vi "From CSV File.vi"(8 "error in (no error)":errorcluster, 9 "Path":path, 10 "engine in":refnum<class "engine configuration.lvclass">, 11 "Scan Engine editor node in":refnum<class "Scan Engine editor node.lvclass">) -> (0 "error out":errorcluster, 1 "Update":bool, 2 "engine out":refnum<class "engine configuration.lvclass">, 3 "Scan Engine editor node out":refnum<class "Scan Engine editor node.lvclass">)   [LabVIEW 2015, in "Scan Engine editor node.lvclass"]
uses:
  Scan Engine editor node.lvclass
  <vilib>/NI/Module Execution Interface/Engine Configuration/engine configuration.lvclass
  configuration/Scan Engine configuration.lvclass
  <vilib>/NI/Configuration Framework/serializable configuration/NISE_CEF_serializable configuration.lvclass/NISE_CEF_serializable configuration.ctl
  configuration/Scan Engine configuration.lvclass/Scan Engine configuration.ctl
  <vilib>/NI/Tag Bus/tag/tag descriptor.lvclass/tag descriptor.ctl
  <vilib>/Utility/LVClass/Get LV Class Name.vi
  <vilib>/NI/Configuration Framework/error generator/NISE_error generator.vi
  <vilib>/NI/Tag Bus Module Framework/channel/TBM channel.lvclass
  <vilib>/NI/Configuration Framework/serializable configuration/NISE_CEF_serializable configuration.lvclass
  <vilib>/NI/Tag Bus/tag/tag descriptor.lvclass
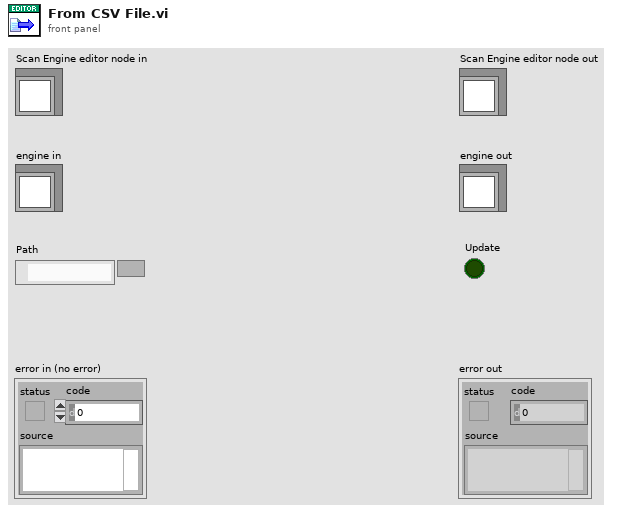
[diagram p1: front panel]
types:
  T1 = typedef "Scan Engine configuration.lvclass/Line.ctl" = cluster{"channel":refnum<class "TBM channel.lvclass">, "Tag":string}
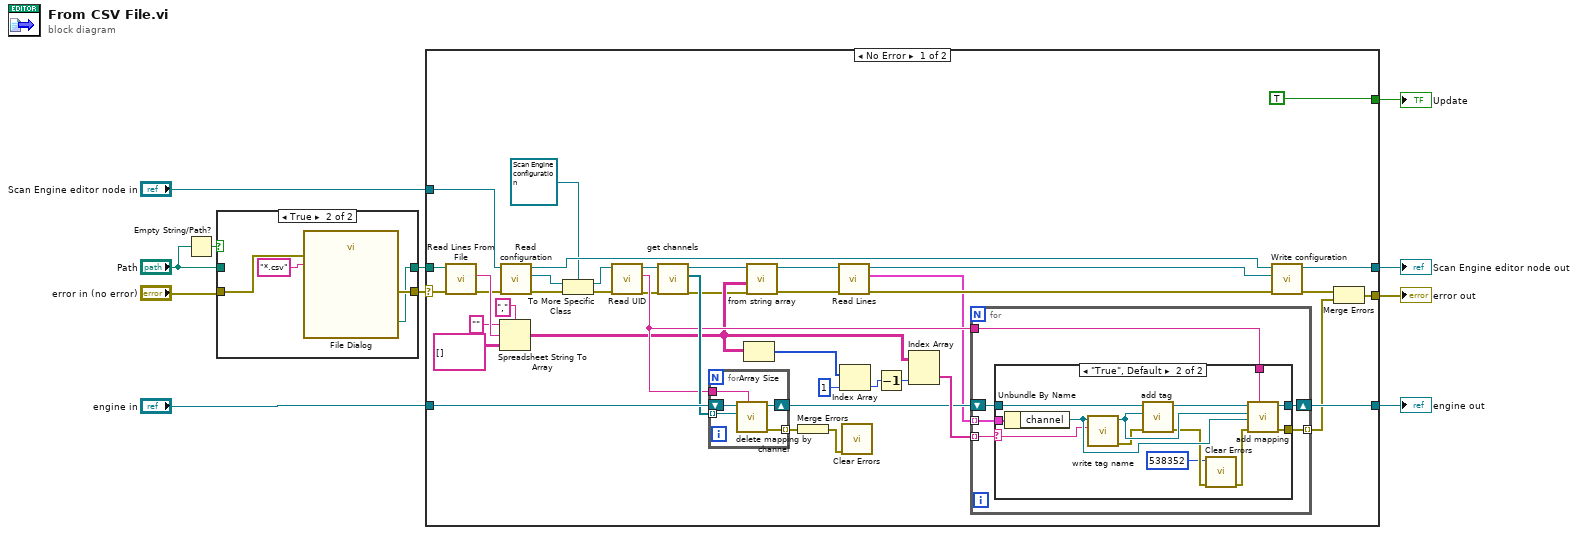
[diagram p0: block diagram]
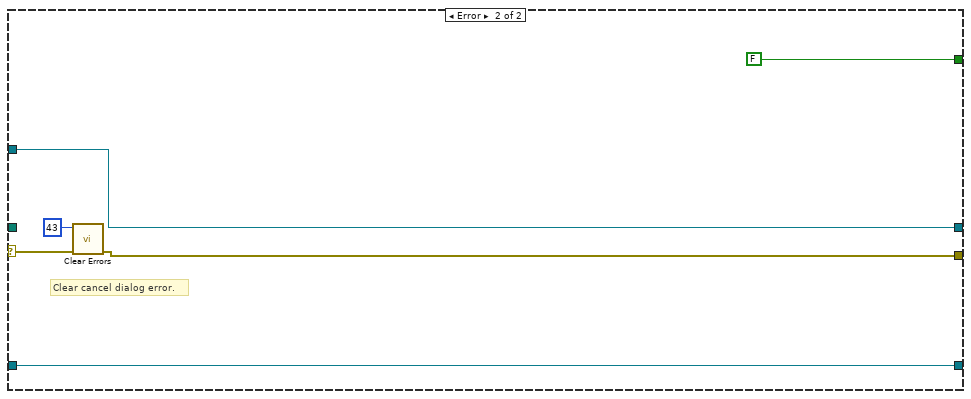
[diagram p4: hidden frame]
diagram:
  n1 = Empty String/Path?(string/path="Path") -> (empty?=w11:bool)
  n2 = case shown="True" w11 {
    tunnel: "error in (no error)" -> [w12 w16]
    tunnel: [w12 w15] -> w5
    tunnel: [w13 w14] -> w6
    tunnel: "Path" -> [w13 _]
    frame False {
    }
    frame True {
      n3 = call "File Dialog"("error in"=w16, "pattern (all files)"="*.csv") -> ("selected path"=w14:path, "error out"=w15:errorcluster)  [unwired: 10 in, 2 out]
    }
  }
  n4 = case shown="No Error" w5 {
    selector: w5 -> [w51 w86]
    tunnel: [w39 w85] -> w1
    tunnel: [w27 w88] -> w4
    tunnel: "Scan Engine editor node in" -> [w32 w88]
    tunnel: w6 -> [w56 _]
    tunnel: [TRUE ("Update") FALSE ("Update")] -> w2
    tunnel: "engine in" -> [w48 w83]
    tunnel: [w41 w83] -> w3
    frame No Error {
      n5 = call <vilib>:"Read Lines From File.vi"("file path (dialog if empty)"=w56, "error in (not an error)"=w51) -> ("line string"=w54:string, "error out"=w31:errorcluster)  [unwired: 5 in, 1 out]
      n6 = Spreadsheet String To Array(delimiter (Tab)=",", format string="", spreadsheet string=w54, array type (2D Dbl)=string[][] [] ("type (empty)")) -> (array=w37:string[][])
      n7 = call-dynamic "Read configuration.vi"("error in"=w31, "Scan Engine editor node in"=w32) -> ("error out"=w29:errorcluster, "configuration"=w30:refnum<class "NISE_CEF_serializable configuration.lvclass">, "Scan Engine editor node out"=w28:refnum<class "Scan Engine editor node.lvclass">)  [unwired: 7 in]
      n8 = To More Specific Class(target class=refnum<class "Scan Engine configuration.lvclass"> refnum ("Scan Engine configuration"), reference=w30, error in=w29) -> (specific class reference=w50:refnum<class "Scan Engine configuration.lvclass">, error out=w44:errorcluster)
      n9 = call <vilib>:"Read UID.vi"("error in"=w44, "configuration in"=w50) -> ("error out"=w24:errorcluster, "instance id"=w40:string, "configuration out"=w49:refnum<class "Scan Engine configuration.lvclass">)  [unwired: 7 in]
      n10 = call-dynamic "get channels.vi"("Scan Engine configuration in"=w49) -> ("channels"=w47:refnum<class "TBM channel.lvclass">[], "Scan Engine configuration out"=w45:refnum<class "Scan Engine configuration.lvclass">)  [unwired: 9 in]
      n11 = for {
        tunnel: w40 -> [w81]
        tunnel: w47 -> [w80] mode=indexing
        tunnel: [w79] -> w46 mode=indexing
        shift-right: [w78] -> w42
        shift-left: w48 -> [w82]
        n12 = call <vilib>:"delete mapping by channel.vi"("owner ID"=w81, "channel"=w80, "engine configuration in"=w82) -> ("error out"=w79:errorcluster, "engine configuration out"=w78:refnum<class "engine configuration.lvclass">)  [unwired: 7 in]
      }
      n13 = Array Size(array=w37) -> (size(s)=w36:i32[])
      n14 = call-dynamic "from string array.vi"("error in (no error)"=w24, "String Array"=w37, "module configuration in"=w45) -> ("error out"=w21:errorcluster, "module configuration out"=w22:refnum<class "Scan Engine configuration.lvclass">)  [unwired: 7 in]
      n15 = Merge Errors(w46) -> (w25:errorcluster)
      n16 = call "Read Lines.vi"("error in (no error)"=w21, "Scan Engine configuration in"=w22) -> ("error out"=w20:errorcluster, "Lines"=w19:T1[], "Scan Engine configuration out"=w18:refnum<class "Scan Engine configuration.lvclass">)  [unwired: 7 in]
      n17 = Index Array(array=w36, index=1) -> (element=w34:i32)
      n18 = call <vilib>:"Clear Errors.vi"("error in (no error)"=w25) -> ()  [unwired: 5 in, 2 out]
      n19 = Decrement(x=w34) -> (x-1=w33:i32)
      n20 = Index Array(array=w37, index (col)=w33) -> (element=w43:string[])  [unwired: 1 in]
      n21 = for {
        tunnel: w19 -> [w63] mode=indexing
        tunnel: w43 -> [w58] mode=indexing
        shift-right: [w62] -> w41
        shift-left: w42 -> [w59]
        tunnel: w40 -> [w61]
        tunnel: [w60] -> w38 mode=indexing
        n22 = case shown="\"True\", Default" w58 {
          selector: w58 -> [_ w65]
          tunnel: w63 -> [_ w77]
          tunnel: [w64 w76] -> w62
          tunnel: w61 -> [_ w75]
          tunnel: [_ w74] -> w60
          tunnel: w59 -> [w64 w73]
          frame "" {
          }
          frame "True", Default {
            n23 = Unbundle By Name(w77) -> ("channel"=w70:refnum<class "TBM channel.lvclass">)
            n24 = call <vilib>:"write tag name.vi"("name"=w65, "system tag in"=w70) -> ("error out"=w69:errorcluster, "system tag out"=w71:refnum<class "TBM channel.lvclass">)  [unwired: 8 in]
            n25 = call-dynamic "add tag.vi"("error in"=w69, "tag descriptor"=w71, "engine configuration in"=w73) -> ("error out"=w68:errorcluster, "engine configuration out"=w72:refnum<class "engine configuration.lvclass">)  [unwired: 7 in]
            n26 = call <vilib>:"Clear Errors.vi"("error in (no error)"=w68, "specific error code to clear (0: all)"=538352) -> ("error out"=w67:errorcluster)  [unwired: 4 in, 1 out]
            n27 = call-dynamic "add mapping.vi"("owner ID"=w75, "error in"=w67, "channel"=w70, "tag descriptor"=w71, "engine configuration"=w72) -> ("error out"=w74:errorcluster, "engine configuration out"=w76:refnum<class "engine configuration.lvclass">)  [unwired: 5 in]
          }
        }
      }
      n28 = call-dynamic "Write configuration.vi"("error in"=w20, "configuration"=w18, "Scan Engine editor node in"=w28) -> ("error out"=w26:errorcluster, "Scan Engine editor node out"=w27:refnum<class "Scan Engine editor node.lvclass">)  [unwired: 7 in]
      n29 = Merge Errors(w26, w38) -> (w39:errorcluster)
    }
    frame Error {
      # "Clear cancel dialog error."
      n30 = call <vilib>:"Clear Errors.vi"("error in (no error)"=w86, "specific error code to clear (0: all)"=43) -> ("error out"=w85:errorcluster)  [unwired: 4 in, 1 out]
    }
  }
  "error out" <- w1
  "Scan Engine editor node out" <- w4
  "Update" <- w2
  "engine out" <- w3
